vi "2Triger Peak detectionM VI.vi"(8 "D Threshold (nA)":dbl format="%#_13g", 9 "U Threshold (nA)":dbl format="%#_13g", 11 "生データの配列":dbl[](array[numeric])=[1.0, 4.0, 3.0, 1.0, 4.0, 1.0, 5.0, 6.0, 7.0, 3.0, 2.0, 1.0, 2.0, 1.0] format="%.4f") -> (0 "Peak Intensity":dbl[](array[numeric]), 2 "Peak#":i32, 3 "Peak location":i32[](array[numeric]), 4 "S End":i32[](array[numeric]), 6 "S Start":i32[](array[numeric]))   [LabVIEW 2018]
panel:
  out "S Peak":i32[](array[numeric])
  out "Graph":dbl[](graph)
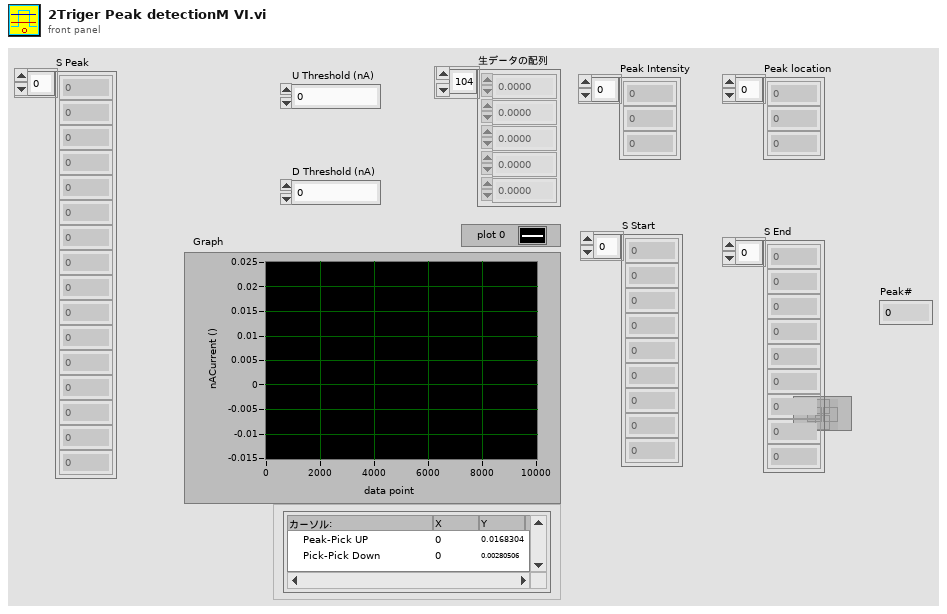
[diagram p1: front panel]
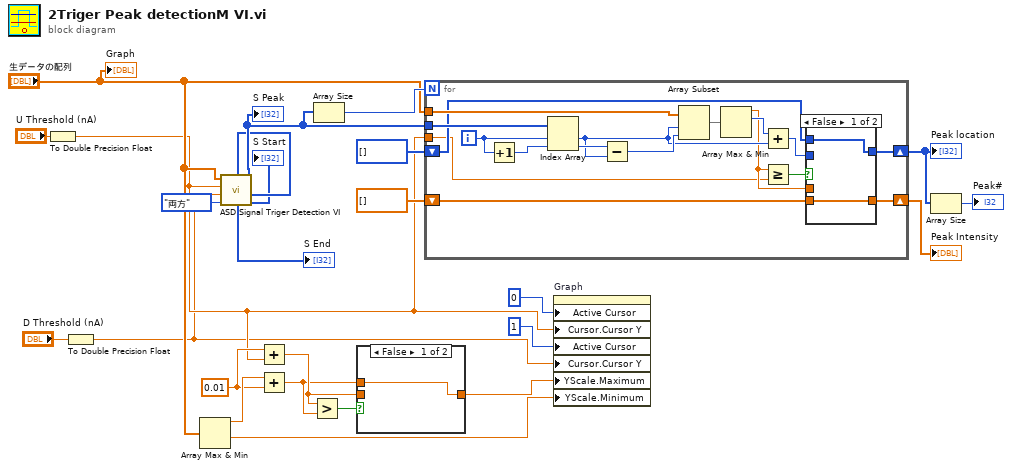
[diagram p0: block diagram]
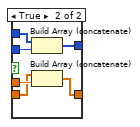
[diagram p3: hidden frame]
diagram:
  w10 = 0.01 ("x")
  n1 = To Double Precision Float(number="U Threshold (nA)") -> (double precision float=w2:dbl)
  n2 = To Double Precision Float(number="D Threshold (nA)") -> (double precision float=w1:dbl)
  n3 = Array Max & Min(array="生データの配列") -> (max value=w14:dbl, min value=w16:dbl)  [unwired: 2 out]
  n4 = call "ASD Signal Triger Detection VI.vi"("方向"=enum16{"両方", "立ち上がり", "立ち下がり"}."両方", "下閾値"=w1, "上閾値"=w2, "入力配列"="生データの配列") -> ("開始"=→"S Start":i32[], "立下り"=→"S End":i32[], "位置"=w5:i32[])  [unwired: 4 in, 1 out]
  "S Peak" <- w5
  n5 = Add(x=w10, y=w2) -> (x+y=w13:dbl)
  n6 = Add(x=w14, y=w10) -> (x+y=w11:dbl)
  n7 = Greater?(x=w13, y=w11) -> (0:w15:bool)
  n8 = Array Size(array=w5) -> (size(s)=w19:i32)
  n9 = case shown="False" w15 {
    tunnel: w13 -> [_ w26]
    tunnel: w11 -> [w25 _]
    tunnel: [w25 w26] -> w12
    frame False {
    }
    frame True {
    }
  }
  n10 = for {
    N: w19 -> [_]
    tunnel: "生データの配列" -> [w42]
    tunnel: w5 -> [w41]
    shift-right: [w36] -> w20
    shift-left: dbl[] [] -> [w35]
    shift-right: [w31] -> w18
    shift-left: i32[] [] -> [w30]
    tunnel: w2 -> [w27]
    i -> [w40]
    n11 = Increment(x=w40) -> (x+1=w39:i32)
    n12 = Index Array(array=w41, index #1=w40, index #2=w39) -> (element #1=w32:i32, element #2=w38:i32)
    n13 = Subtract(x=w38, y=w32) -> (x-y=w43:i32)
    n14 = Array Subset(array=w42, index=w32, length=w43) -> (w37:dbl[])
    n15 = Array Max & Min(array=w37) -> (max value=w28:dbl, max index (indices)=w34:i32)  [unwired: 2 out]
    n16 = Add(x=w34, y=w32) -> (x+y=w33:i32)
    n17 = Greater Or Equal?(x=w28, y=w27) -> (x >= y?=w29:bool)
    n18 = case shown="False" w29 {
      tunnel: w28 -> [_ w51]
      tunnel: [w45 w50] -> w36
      tunnel: w35 -> [w45 w49]
      tunnel: w33 -> [_ w48]
      tunnel: [w44 w47] -> w31
      tunnel: w30 -> [w44 w46]
      frame False {
      }
      frame True {
        n19 = Build Array (concatenate)(w46, w48) -> (w47:i32[])
        n20 = Build Array (concatenate)(w49, w51) -> (w50:dbl[])
      }
    }
  }
  "Peak Intensity" <- w20
  "Peak location" <- w18
  n21 = property on="Graph" class="WFGraph (strict)"("Active Cursor"=u32 0 ("アクティブカーソル"), "Cursor.Cursor Y"=w2, "Active Cursor"=u32 1 ("アクティブカーソル"), "Cursor.Cursor Y"=w1, "YScale.Maximum"=w12, "YScale.Minimum"=w16) -> ()  [unwired: 2 in, 2 out]
  n22 = Array Size(array=w18) -> (size(s)=→"Peak#":i32)
  "Graph" <- "生データの配列"
